vi "Own20261012_GetStructureInfo.vi"() -> ()   [LabVIEW 2024]
panel:
  out "error out":errorcluster caption="错误输出"
  out "tunnel_ids":refnum<vi>[](array[refnum])
  out "diagram_ids":refnum<vi>[](array[refnum])
  out "owner_id":refnum<vi>
  in  "structure_id":u32
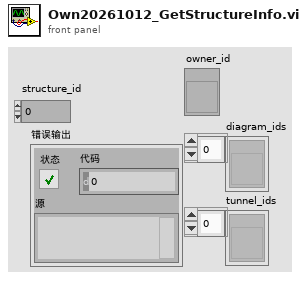
[diagram p1: front panel]
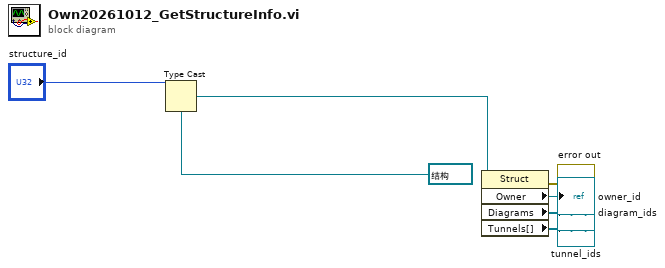
[diagram p0: block diagram]
diagram:
  n1 = Type Cast(type=refnum<vi> refnum ("引用"), x="structure_id") -> (*(type *) &x=w5:refnum<vi>)
  n2 = property class="Struct"(reference=w5) -> (error out=→"error out":errorcluster, "Owner"=→"owner_id":refnum<vi>, "Diagrams"=→"diagram_ids":refnum<vi>[], "Tunnels[]"=→"tunnel_ids":refnum<vi>[])  [unwired: 1 in, 1 out]
